vi "GOOP_UMLEditor_CallMain.vi"(0 "AppRef":refnum<vi>, 1 "Enum":T1, 2 "Project":string, 3 "Class/VI-Path":path, 4 "Target":string, 5 "error in (no error)":errorcluster) -> (19 "error out":errorcluster)   [LabVIEW 2020]
uses:
  GOOP_UMLEditor_CallMainAction.ctl
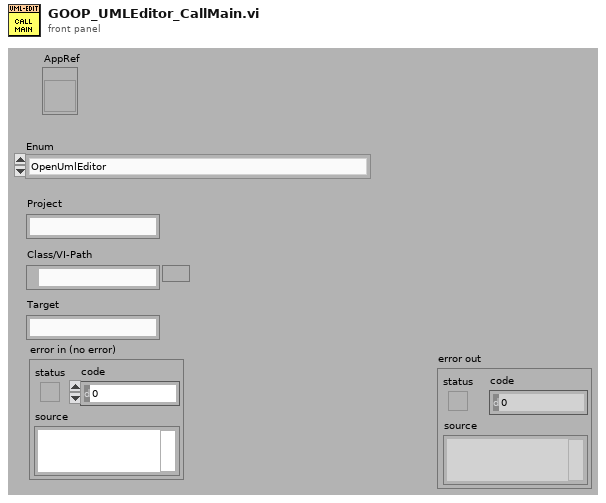
[diagram p1: front panel]
types:
  T1 = typedef "GOOP_UMLEditor_CallMainAction.ctl" = enum16{"OpenUmlEditor", "ReverseEngineering:WholeProject", "ReverseEngineering:OneClass", "ReverseEngineering:OneVI", "ShowInStateDiagram:OneVI", "OpenUMLFile"}
  T2 = enum32{"Bad", "Idle", "Run top level", "Running"}
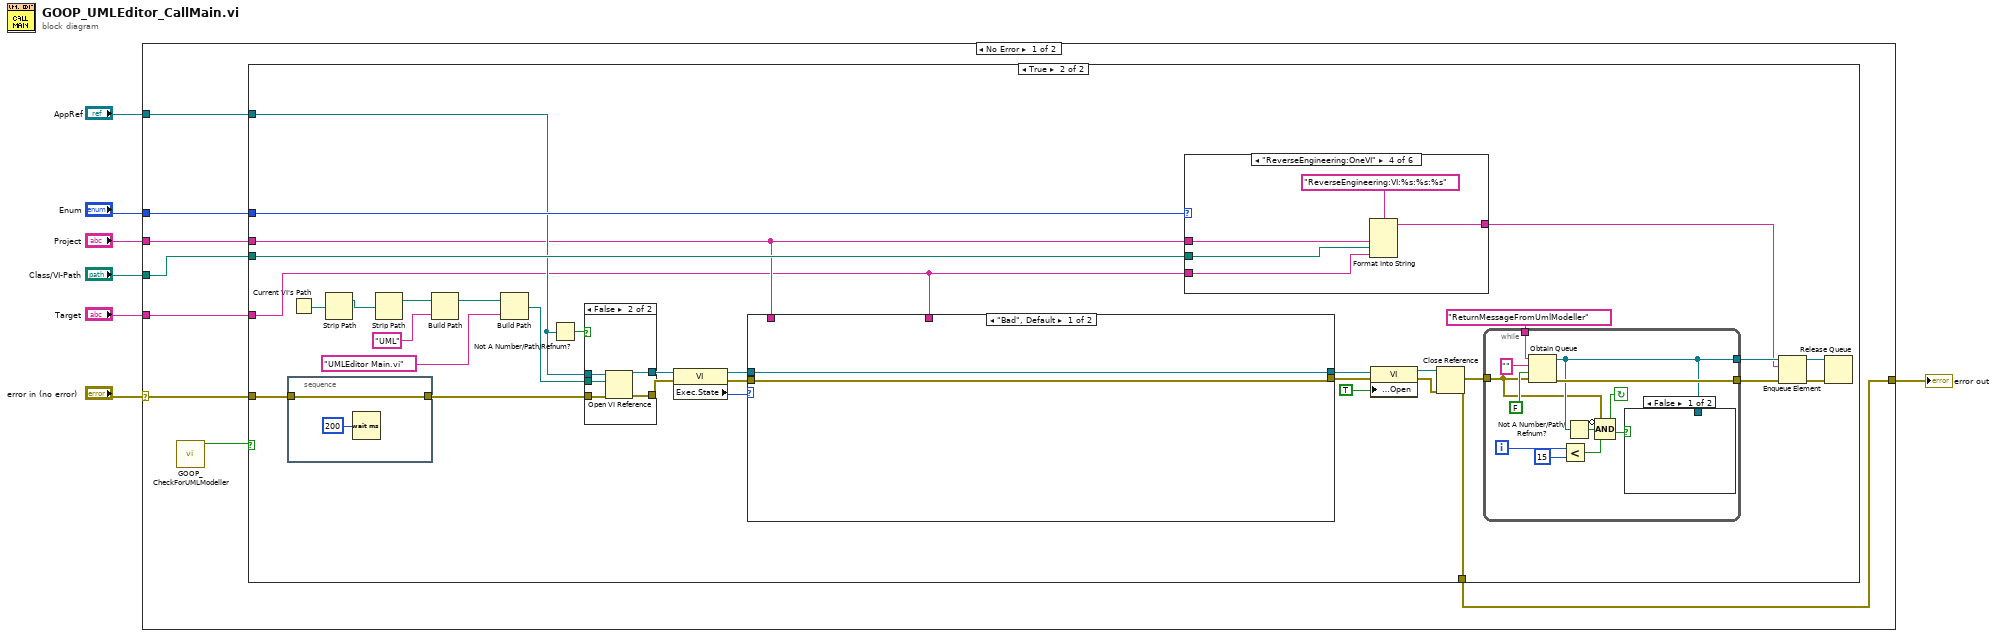
[diagram p0: block diagram]
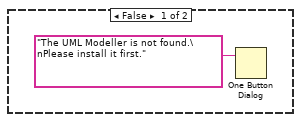
[diagram p2: hidden frame]
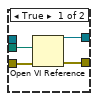
[diagram p3: hidden frame]
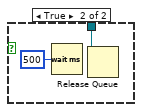
[diagram p4: hidden frame]
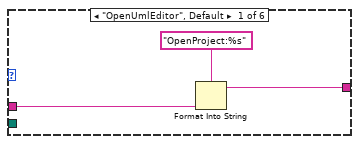
[diagram p5: hidden frame]
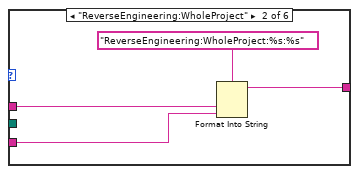
[diagram p6: hidden frame]
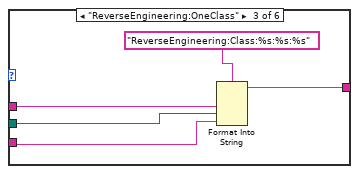
[diagram p7: hidden frame]
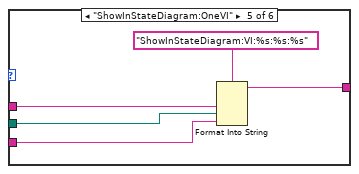
[diagram p8: hidden frame]
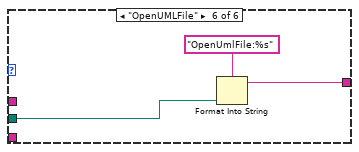
[diagram p9: hidden frame]
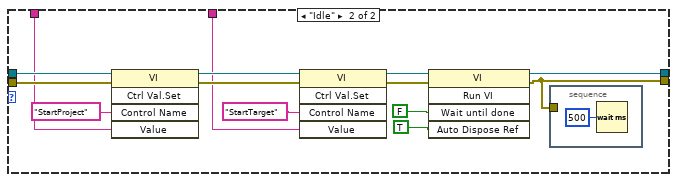
[diagram p10: hidden frame]
diagram:
  n1 = case shown="No Error" "error in (no error)" {
    selector: "error in (no error)" -> [w13 w115]
    tunnel: "Enum" -> [w15 _]
    tunnel: [w12 w115] -> w5
    tunnel: "Project" -> [w10 _]
    tunnel: "Class/VI-Path" -> [w14 _]
    tunnel: "AppRef" -> [w11 _]
    tunnel: "Target" -> [w9 _]
    frame No Error {
      n2 = call "GOOP_CheckForUMLModeller.vi"() -> ("UML Modeller Exists"=w8:bool)  [unwired: 10 in, 1 out]
      n3 = case shown="True" w8 {
        tunnel: w15 -> [_ w33]
        tunnel: w14 -> [_ w26]
        tunnel: w13 -> [_ w25]
        tunnel: [_ w21] -> w12
        tunnel: w11 -> [_ w19]
        tunnel: w10 -> [_ w18]
        tunnel: w9 -> [_ w17]
        frame False {
          n4 = One Button Dialog(message="The UML Modeller is not found.\nPlease install it first.") -> ()  [unwired: 1 in, 1 out]
        }
        frame True {
          n5 = stacked-sequence {
            tunnel: [w59] -> w24
            tunnel: w25 -> [w59]
            frame #0 {
              n6 = Wait (ms)(milliseconds to wait=u32 200) -> ()  [unwired: 1 out]
            }
          }
          n7 = Current VI's Path() -> (path=w48:path)
          n8 = Strip Path(path=w48) -> (stripped path=w47:path)  [unwired: 1 out]
          n9 = Strip Path(path=w47) -> (stripped path=w46:path)  [unwired: 1 out]
          n10 = Build Path(base path=w46, name or relative path="UML") -> (appended path=w44:path)
          n11 = Build Path(base path=w44, name or relative path="UMLEditor Main.vi") -> (appended path=w42:path)
          n12 = Not A Number/Path/Refnum?(number/path/refnum=w19) -> (NaN/Path/Refnum?=w20:bool)
          n13 = case shown="False" w20 {
            tunnel: w42 -> [w52 w57]
            tunnel: [w51 w56] -> w41
            tunnel: [w50 w55] -> w40
            tunnel: w24 -> [w49 w54]
            tunnel: w19 -> [_ w53]
            frame True {
              n14 = Open VI Reference(vi path=w52, error in (no error)=w49) -> (vi reference=w51:refnum<vi>, error out=w50:errorcluster)  [unwired: 4 in]
            }
            frame False {
              n15 = Open VI Reference(application reference (local)=w53, vi path=w57, error in (no error)=w54) -> (vi reference=w56:refnum<vi>, error out=w55:errorcluster)  [unwired: 3 in]
            }
          }
          n16 = property class="VI"(reference=w41, error in=w40) -> (reference out=w38:refnum<vi>, error out=w37:errorcluster, "Exec.State"=w39:T2)
          n17 = case shown="\"Bad\", Default" w39 {
            tunnel: w38 -> [w99 w109]
            tunnel: w37 -> [w98 w108]
            tunnel: [w99 w112] -> w36
            tunnel: [w98 w110] -> w35
            tunnel: w18 -> [_ w106]
            tunnel: w17 -> [_ w100]
            frame "Bad", Default {
            }
            frame "Idle" {
              n18 = invoke class="VI" method="Ctrl Val.Set"(reference=w109, error in=w108, "Control Name"="StartProject", "Value"=w106) -> (reference out=w105:refnum<vi>, error out=w104:errorcluster)  [unwired: 1 in, 3 out]
              n19 = invoke class="VI" method="Ctrl Val.Set"(reference=w105, error in=w104, "Control Name"="StartTarget", "Value"=w100) -> (reference out=w101:refnum<vi>, error out=w102:errorcluster)  [unwired: 1 in, 3 out]
              n20 = invoke class="VI" method="Run VI"(reference=w101, error in=w102, "Wait until done"=FALSE ("Wait Until Done"), "Auto Dispose Ref"=TRUE ("Front Panel Window:Open")) -> (reference out=w112:refnum<vi>, error out=w110:errorcluster)  [unwired: 1 in, 3 out]
              n21 = stacked-sequence {
                tunnel: w110 -> [_]
                frame #0 {
                  n22 = Wait (ms)(milliseconds to wait=u32 500) -> ()  [unwired: 1 out]
                }
              }
            }
          }
          n23 = case shown="\"ReverseEngineering:OneVI\"" w33 {
            tunnel: w18 -> [w74 w78 w83 w88 w93 _]
            tunnel: [w73 w77 w82 w87 w92 w96] -> w27
            tunnel: w26 -> [_ _ w81 w86 w91 w95]
            tunnel: w17 -> [_ w76 w80 w85 w90 _]
            frame "OpenUmlEditor", Default {
              n24 = Format Into String(format string="OpenProject:%s", w74) -> (resulting string=w73:string)  [unwired: 2 in, 1 out]
            }
            frame "ReverseEngineering:WholeProject" {
              n25 = Format Into String(format string="ReverseEngineering:WholeProject:%s:%s", w78, w76) -> (resulting string=w77:string)  [unwired: 2 in, 1 out]
            }
            frame "ReverseEngineering:OneClass" {
              n26 = Format Into String(format string="ReverseEngineering:Class:%s:%s:%s", w83, w81, w80) -> (resulting string=w82:string)  [unwired: 2 in, 1 out]
            }
            frame "ReverseEngineering:OneVI" {
              n27 = Format Into String(format string="ReverseEngineering:VI:%s:%s:%s", w88, w86, w85) -> (resulting string=w87:string)  [unwired: 2 in, 1 out]
            }
            frame "ShowInStateDiagram:OneVI" {
              n28 = Format Into String(format string="ShowInStateDiagram:VI:%s:%s:%s", w93, w91, w90) -> (resulting string=w92:string)  [unwired: 2 in, 1 out]
            }
            frame "OpenUMLFile" {
              n29 = Format Into String(format string="OpenUmlFile:%s", w95) -> (resulting string=w96:string)  [unwired: 2 in, 1 out]
            }
          }
          n30 = property class="VI"(reference=w36, error in=w35, "Front Panel.Open"=TRUE ("Front Panel Window:Open")) -> (reference out=w23:refnum<vi>, error out=w22:errorcluster)
          n31 = Close Reference(reference=w23, error in (no error)=w22) -> (error out=w21:errorcluster)
          n32 = while {
            tunnel: "ReturnMessageFromUmlModeller" ("name (unnamed)") -> [w70]
            tunnel: [w61] -> w31
            tunnel: [w62] -> w30
            tunnel: w21 -> [w60]
            i -> [w68]
            stop <- w65 continue-if-true
            n33 = Obtain Queue(name (unnamed)=w70, element data type="", create if not found? (T)=FALSE, error in (no error)=w60) -> (queue out=w61:refnum<queue>, error out=w62:errorcluster)  [unwired: 1 in, 1 out]
            n34 = Less?(x=w68, y=15) -> (x < y?=w66:bool)
            n35 = Not A Number/Path/Refnum?(number/path/refnum=w61) -> (NaN/Path/Refnum?=w67:bool)
            n36 = Compound Arithmetic op=AND(invert w60, w67, w66) -> (w65:bool)
            n37 = case shown="False" w65 {
              tunnel: w61 -> [_ w71]
              frame False {
              }
              frame True {
                n38 = Wait (ms)(milliseconds to wait=u32 500) -> ()  [unwired: 1 out]
                n39 = Release Queue(queue=w71) -> ()  [unwired: 2 in, 3 out]
              }
            }
          }
          n40 = Enqueue Element(queue=w31, element=w27, error in (no error)=w30) -> (queue out=w29:refnum<queue>, error out=w28:errorcluster)  [unwired: 1 in, 1 out]
          n41 = Release Queue(queue=w29, error in (no error)=w28) -> ()  [unwired: 1 in, 3 out]
        }
      }
    }
    frame Error {
    }
  }
  "error out" <- w5
